vi "Get_MultiVar_Value.vi"(8 "error in (no error)":errorcluster, 10 "varName":string, 11 "muExpr in":refnum<class "mupExpr.lvclass">) -> (0 "error out":errorcluster, 2 "Value":dbl, 3 "muExpr out":refnum<class "mupExpr.lvclass">)   [LabVIEW 2015, in "mupExpr.lvclass"]
doc: "Lookup variable value by name."
uses:
  mupExpr.lvclass
  mupExpr.lvclass/mupExpr.ctl
  <vilib>/Utility/error.llb/Error Cluster From Error Code.vi
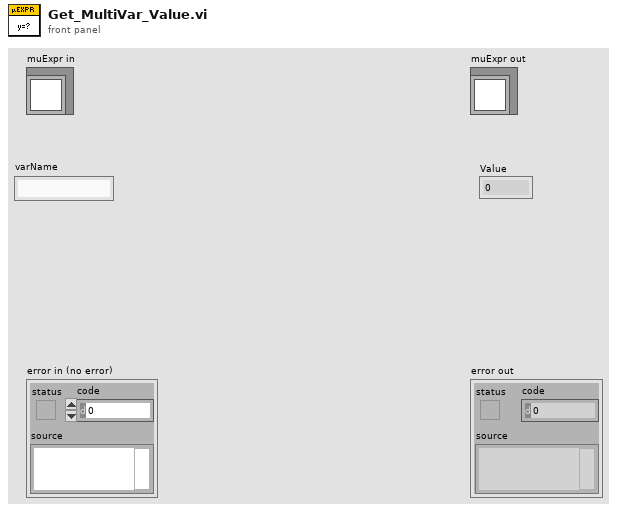
[diagram p1: front panel]
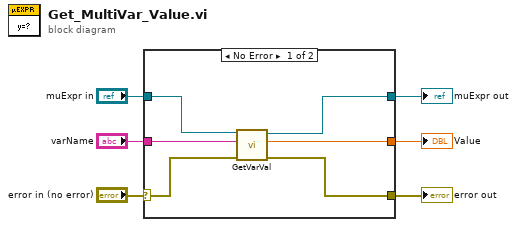
[diagram p0: block diagram]
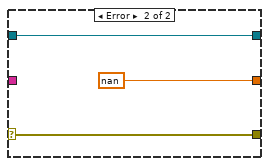
[diagram p2: hidden frame]
diagram:
  n1 = case shown="No Error" "error in (no error)" {
    selector: "error in (no error)" -> [w10 w15]
    tunnel: [w9 w15] -> w5
    tunnel: [w7 w14] -> w3
    tunnel: "muExpr in" -> [w8 w14]
    tunnel: [w12 nan ("pd")] -> w2
    tunnel: "varName" -> [w11 _]
    frame No Error {
      n2 = call "GetVarVal.vi"("error in (no error)"=w10, "varName"=w11, "muExpr in"=w8) -> ("error out"=w9:errorcluster, "varValue"=w12:dbl, "muExpr out"=w7:refnum<class "mupExpr.lvclass">)  [unwired: 6 in]
    }
    frame Error {
    }
  }
  "error out" <- w5
  "muExpr out" <- w3
  "Value" <- w2
